vi "Linear Measurement.vi"() -> ()   [LabVIEW 2020, in "Data Viewer.lvlib"]
uses:
  Data Viewer.lvlib
panel:
  out "Y2":dbl
  out "X2":dbl
  out "Y1":dbl
  out "X1":dbl
  in  "CMDQ":refnum<queue>
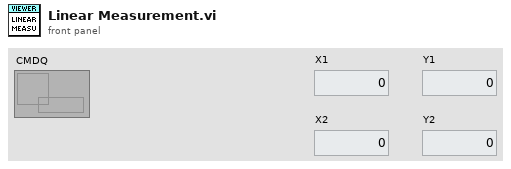
[diagram p1: front panel]
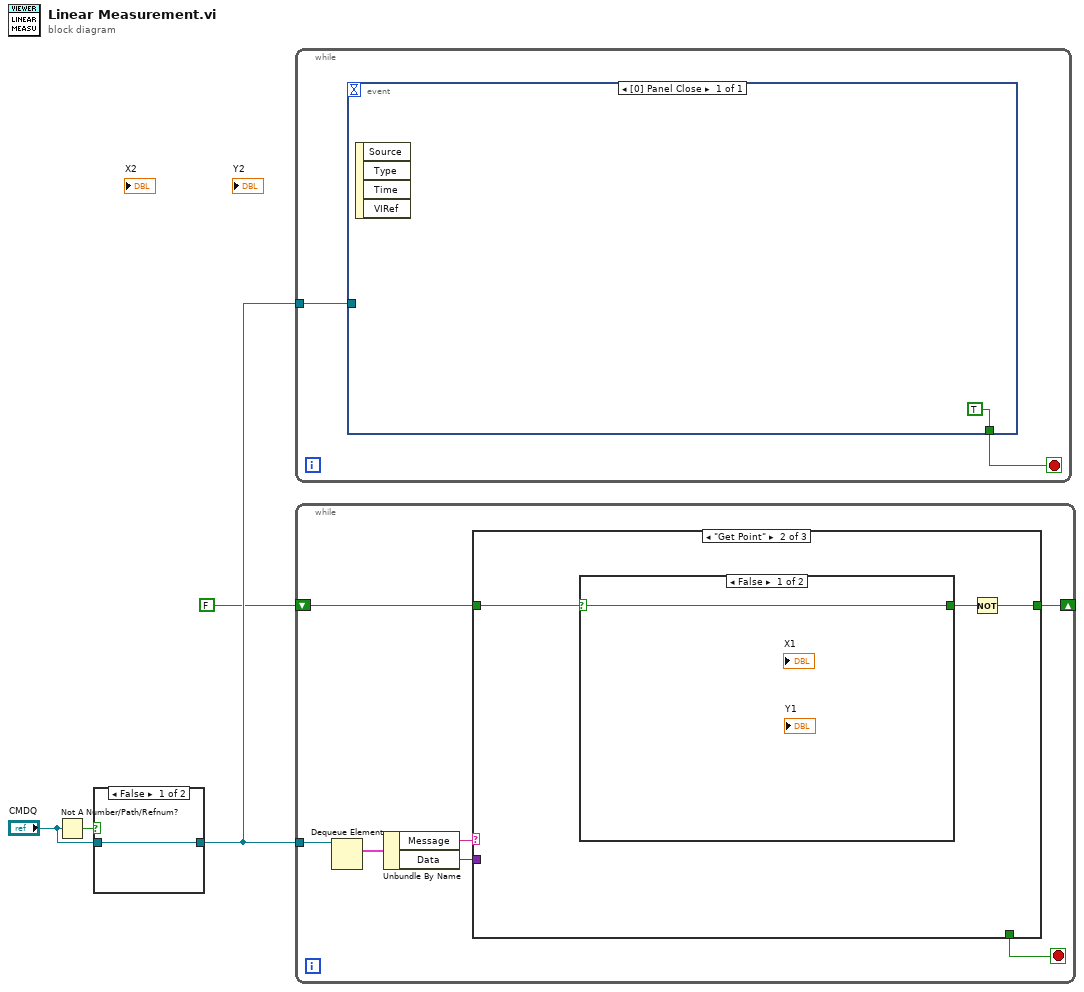
[diagram p0: block diagram]
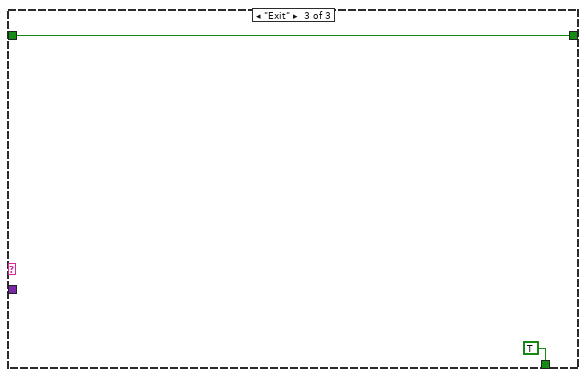
[diagram p4: hidden frame]
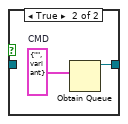
[diagram p5: hidden frame]
diagram:
  n1 = Not A Number/Path/Refnum?(number/path/refnum="CMDQ") -> (NaN/Path/Refnum?=w4:bool)
  n2 = case shown="False" w4 {
    tunnel: [w5 w6] -> w3
    tunnel: "CMDQ" -> [w5 _]
    frame False {
    }
    frame True {
      w7 = cluster{"Message":string, "Data":variant} {"Message"="", "Data"=variant}  # CMD
      n3 = Obtain Queue(element data type=w7) -> (queue out=w6:refnum<queue>)  [unwired: 4 in, 2 out]
    }
  }
  n4 = while {
    tunnel: w3 -> [w8]
    stop <- w9 stop-if-true
    n5 = event shown="[0] Panel Close" {
      selector: _ -> [_]
      dyn-events: _ -> [_]
      timeout: _ -> [_]
      tunnel: [TRUE] -> w9
      tunnel: w8 -> [_]
      event Panel Close {
        n6 = event-data() -> ()  [unwired: 1 in, 4 out]
      }
    }
  }
  n7 = while {
    tunnel: w3 -> [w17]
    shift-right: [w12] -> _
    shift-left: FALSE -> [w11]
    stop <- w13 stop-if-true
    n8 = Dequeue Element(queue=w17) -> (element=w16:cluster{"Message":string, "Data":variant})  [unwired: 2 in, 3 out]
    n9 = Unbundle By Name(w16) -> ("Message"=w15:string, "Data"=w14:variant)
    n10 = case shown="\"Get Point\"" w15 {
      tunnel: w14 -> [_ _ _]
      tunnel: [_ _ TRUE] -> w13
      tunnel: [w18 w19 w24] -> w12
      tunnel: w11 -> [w18 w21 w24]
      frame "假", Default {
      }
      frame "Get Point" {
        n11 = case shown="False" w21 {
          selector: w21 -> [w22 w23]
          tunnel: [w22 w23] -> w20
          frame False {
          }
          frame True {
          }
        }
        n12 = Not(x=w20) -> (.not. x?=w19:bool)
      }
      frame "Exit" {
      }
    }
  }
